vi "Fo-Epc-In.vi"(1 "As (Area del OLED) m2":dbl, 4 "S (Distancia OLED-fotodiodo) m":dbl, 6 "Color":T1 items=["Violeta(360-450nm)", "Azul(450-500nm)", "Verde (500-570nm)", "Amarillo (570-590nm)", "Naranja (590-610)", "Rojo (610-670nm)", "Blanco"]) -> (14 "Iluminancia (lm/m2)":dbl, 15 "Pin":dbl, 17 "Analog Vout":dbl, 19 "Luminancia (Cd/m2)":dbl)   [LabVIEW 2020]
uses:
  controls/Color --typedef.ctl
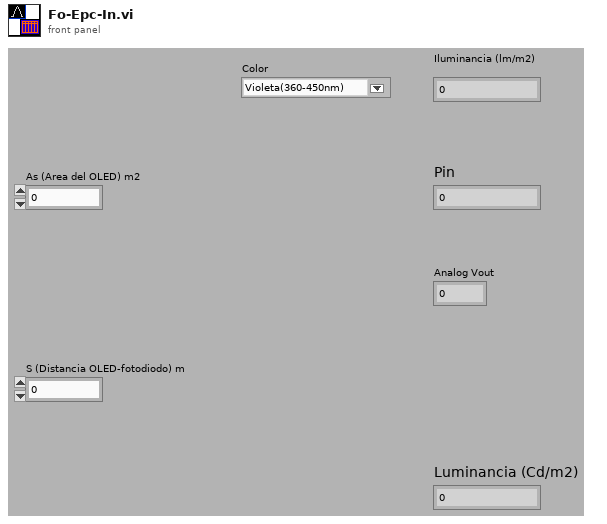
[diagram p1: front panel]
types:
  T1 = typedef "Color --typedef.ctl" = u16
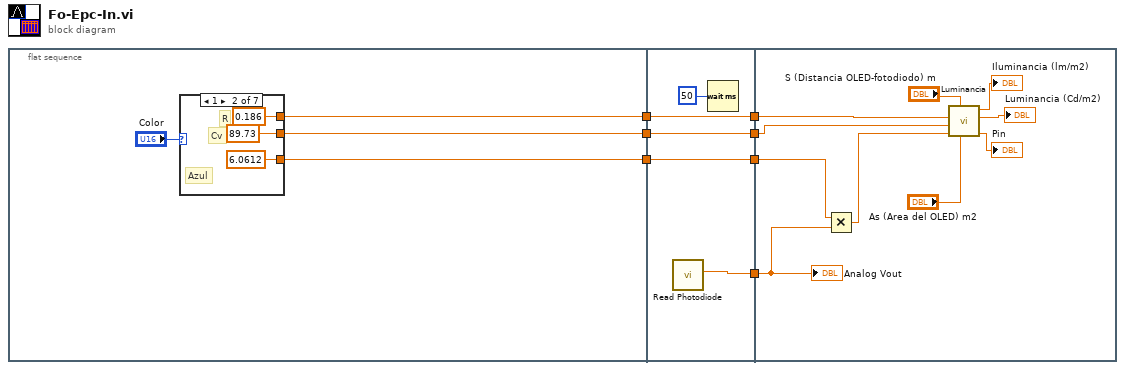
[diagram p0: block diagram]
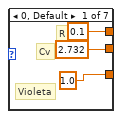
[diagram p2: hidden frame]
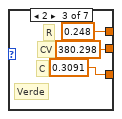
[diagram p3: hidden frame]
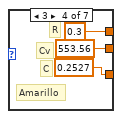
[diagram p4: hidden frame]
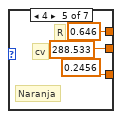
[diagram p5: hidden frame]
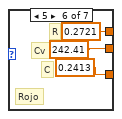
[diagram p6: hidden frame]
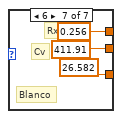
[diagram p7: hidden frame]
diagram:
  n1 = flat-sequence {
    tunnel: [w10] -> w7
    tunnel: [w9] -> w6
    tunnel: [w8] -> w2
    tunnel: [w37] -> w5
    tunnel: [w36] -> w4
    tunnel: w7 -> [w36]
    tunnel: w6 -> [w35]
    tunnel: [w35] -> w3
    tunnel: w2 -> [w33]
    tunnel: [w33] -> w1
    tunnel: w5 -> [w40]
    tunnel: w4 -> [w43]
    tunnel: w3 -> [w42]
    tunnel: w1 -> [w38]
    frame #0 {
      n2 = case shown="1" "Color" {
        tunnel: [0.1 0.186 0.248 0.3 0.646 0.2721 0.256] -> w10
        tunnel: [2.732 89.73 380.298 553.56 288.533 242.41 411.91] -> w9
        tunnel: [1.0 6.0612 0.3091 0.2527 0.2456 0.2413 26.582] -> w8
        frame 0, Default {
          # "Violeta"
          # "Cv"
          # "R"
        }
        frame 1 {
          # "Azul"
          # "Cv"
          # "R"
        }
        frame 2 {
          # "C"
          # "Verde"
          # "CV"
          # "R"
        }
        frame 3 {
          # "C"
          # "Amarillo"
          # "Cv"
          # "R"
        }
        frame 4 {
          # "Naranja"
          # "cv"
          # "R"
        }
        frame 5 {
          # "C"
          # "Rojo"
          # "Cv"
          # "R"
        }
        frame 6 {
          # "Blanco"
          # "Cv"
          # "Rx"
        }
      }
    }
    frame #1 {
      n3 = call "Read Photodiode.vi"() -> ("Analog  Vout"=w37:dbl)  [unwired: 2 in, 9 out]
      n4 = Wait (ms)(milliseconds to wait=u32 50) -> ()  [unwired: 1 out]
    }
    frame #2 {
      n5 = Multiply(x=w38, y=w40) -> (x*y=w39:dbl)
      n6 = call "Luminancia.vi"("As (Area del OLED) cm2"="As (Area del OLED) m2", "S (Distancia OLED-fotodiodo) cm"="S (Distancia OLED-fotodiodo) m", "Analog Vout"=w39, "Respuesta futopica (Cv)"=w42, "Responsividad Normalizada (R)"=w43) -> ("Pin(W)"=→"Pin":dbl, "Luminancia (Cd/m2)"=→"Luminancia (Cd/m2)":dbl, "Iluminancia  lm/m2"=→"Iluminancia (lm/m2)":dbl)  [unwired: 3 out]
      "Analog Vout" <- w40
    }
  }
